vi "PicoScope4000Close.vi"(8 "error in (no error)":errorcluster, 11 "handle":i16) -> (0 "error out":errorcluster)   [LabVIEW 2009]
doc: "This closes the oscilloscope and should be called before exiting an application."
uses:
  ps4000.dll
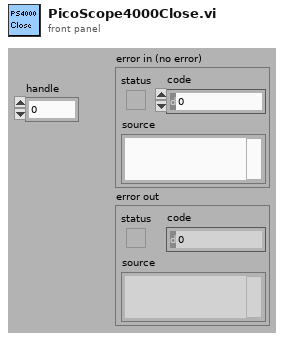
[diagram p1: front panel]
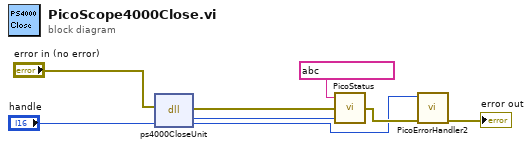
[diagram p0: block diagram]
diagram:
  n1 = dll-call lib="ps4000.dll" fn="ps4000CloseUnit" ("ps3000.dll:_ps3000_open_unit@0")(error in="error in (no error)", "handle"="handle") -> (error out=w4:errorcluster, "PICO_STATUS"=w3:u32, "handle"=w2:i16)  [unwired: 2 in, 1 out]
  n2 = call "PicoStatus.vi"("PICO STATUS"=w3, "error in"=w4, "source"=string ?) -> ("error out"=w5:errorcluster)
  n3 = call "PicoErrorHandler2.vi"("error in (no error)"=w5, "handle In"=w2) -> ("error out"=→"error out":errorcluster)  [unwired: 9 in]
